vi "Client Tests.vi"() -> ()   [LabVIEW 2025]
uses:
  controls/Clint States Tests.ctl
  5TR Lab/5TR Lab/Global Variables/cRIO channels Input.vi
  5TR Lab/5TR Lab/Global Variables/General Glob.vi
panel:
  in  "Seek Forward Button":bool
  in  "Tab Control 3":T1(tab)
  in  "Cluster":T2
  in  "Cluster 2":T3
  in  "ID_HEATER_Stage_3 2":bool
  in  "ID_HEATER_Stage_2 2":bool
  in  "OD_HEATER_Stage_1":bool
  in  "ID_HEATER_Stage_3":bool
  in  "ID_HEATER_Stage_2":bool
  in  "Cluster 3":T4
  in  "AUX Chiller Pump_ 2":bool
  in  "AUX Chiller Pump_1":bool
  in  "Hc0 2":i32(listbox)
  out "Type Of Test":string
  in  "Add paramter":bool
  in  "Hc0":i32(listbox)
  out "Temp\n(C)":T5 {"UUT Discharge temp" format="%0.2f"; "UUT Suction temp" format="%0.2f"; "UUT Liquid temp" format="%0.2f"}
  out "Pressures\n(Mpa)":T6 {"UUT Discharge Pressure" format="%0.2f"; "UUT Suction Pressure" format="%0.2f"; "UUT Liquid Pressure" format="%0.2f"}
  in  "Tab Control":enum32{"Water Side capacity", "Page 2"}(tab)
  in  "Tab Control 2":T7(tab)
  out "WFR":dbl format="%0.2f"
  out "WPD":dbl format="%0.2f"
  out "T. Diff":dbl format="%0.2f"
  out "LWT":dbl format="%0.2f"
  out "EWT":dbl format="%0.2f"
  out "Running 3":bool
  out "Water Capacity":dbl format="%0.2f"
  out "Latent Capacity":dbl format="%0.2f"
  out "Sensible Capacity":dbl format="%0.2f"
  out "ID Entering WB":dbl format="%0.2f"
  out "ID Entering DB":dbl format="%0.2f"
  out "ID Leaving WB":dbl format="%0.2f"
  out "ID Leaving DB":dbl format="%0.2f"
  out "Air Capacity W":dbl format="%0.1f"
  out "Running 2":bool
  out "HB 2":dbl format="%0.2f"
  out "Running":bool
  out "Heat Balance %":dbl format="%0.1f"
  out "SC":dbl format="%0.2f"
  out "SH":dbl format="%0.2f"
  out "UUT Liquid Pressure 2":dbl format="%0.2f"
  out "Running":bool
  in  "Refrigerant":enum16{"R407c", "R410a", "R134a", "R22", ""}(ring)
  in  "Running Tests":string[](array[string])
  out "Total Capacity ID":dbl format="%0.2f"
  out "Total Capacity OD":dbl format="%0.2f"
  out "HB":dbl format="%0.2f"
  out "ID WFR":dbl format="%0.1f"
  out "result":dbl
  # "Sensor I/P Readings"
  # "Sensor O/P Values"
  # "W/W"
  # "Total Capacity\nWater-Side"
  # "C"
  # "C"
  # "C"
  # "gpm"
  # "Psi"
  # "Total Capacity\n Air-Side"
  # "DBT"
  # "WBT"
  # "Return"
  # "Supply"
  # "W"
  # "W"
  # "W"
  # "%"
  # "Thermal Transmittance"
  # "Thermal Bridging"
  # "Refrigerant"
  # "C"
  # "C"
  # "Ref Capacity"
  # "W"
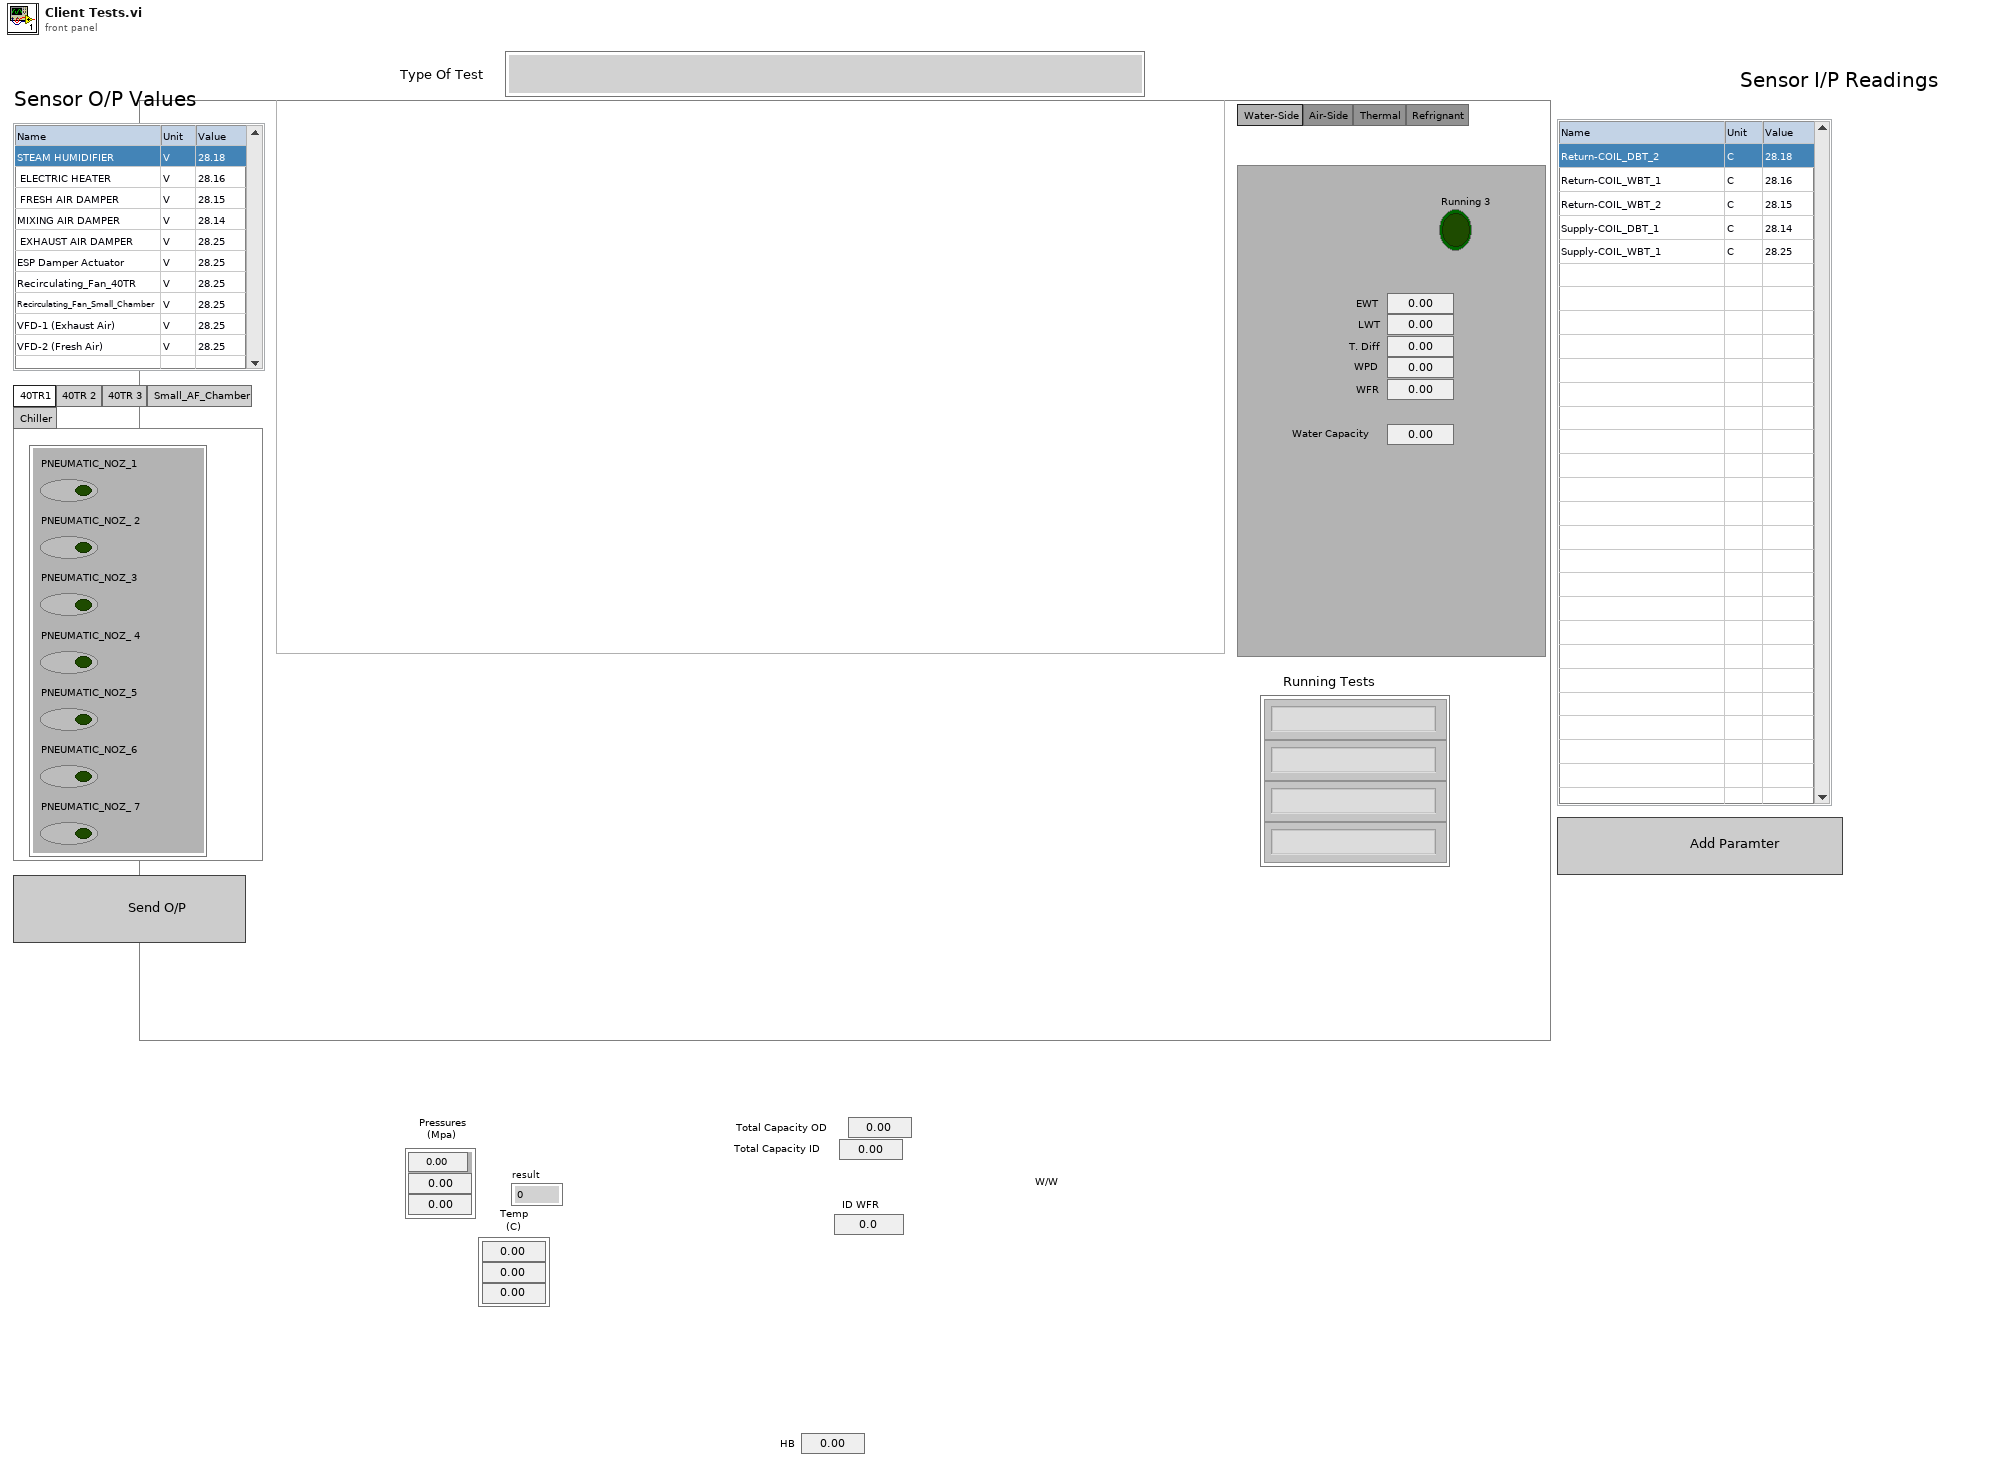
[diagram p1: front panel]
types:
  T1 = enum32{"40TR1", "40TR 2", "40TR 3", "Small_AF_Chamber", "Chiller"}
  T2 = cluster{"PNEUMATIC_NOZ_1":bool, "PNEUMATIC_NOZ_ 2":bool, "PNEUMATIC_NOZ_3":bool, "PNEUMATIC_NOZ_ 4":bool, "PNEUMATIC_NOZ_5":bool, "PNEUMATIC_NOZ_6":bool, "PNEUMATIC_NOZ_ 7":bool}
  T3 = cluster{"Recirculating_Fan_40TR":bool, "Recirculating_Fan_40TR 2":bool, "STEAM HUMIDIFIER":bool, "VFD-2 (Exahust Air)":bool, "VFD-2 (Fresh Air) ":bool, "VFD_Fan_Leak_setup":bool, "ID_HEATER_Stage_1":bool}
  T4 = cluster{"PNEUMATIC_NOZ_1":bool, "PNEUMATIC_NOZ_ 2":bool, "PNEUMATIC_NOZ_3":bool, "PNEUMATIC_NOZ_ 4":bool, "PNEUMATIC_NOZ_5":bool}
  T5 = cluster{"UUT Liquid temp":dbl, "UUT Suction temp":dbl, "UUT Discharge temp":dbl}
  T6 = cluster{"UUT Liquid Pressure":dbl, "UUT Suction Pressure":dbl, "UUT Discharge Pressure":dbl}
  T7 = enum32{"Water-Side", "Air-Side", "Thermal", "Refrignant"}
  T8 = typedef "Clint States Tests.ctl" = enum16{"Initialize", "Water Side", "Sensible capacity", "AIR SIDE Capacity", "Refrigrator Capacity"}
  T9 = cluster{"Room DP":dbl, "Barometric Pressure":dbl, "ID Nozzle DP":dbl, "OD Nozzle DP":dbl, "OD UUT Discharge Pressure":dbl, "OD UUT Suction Pressure":dbl, "OD UUT Liquid Pressure":dbl, "ID Humidifier Weight ":dbl, "ID UUT Condensate Weight":dbl, "ID Coil Condensate Weight":dbl, "OD Coil Water flow rate":dbl, "ID Flow Meter Channel":dbl}
  T10 = cluster{"ID UUT inlet DBT":dbl, "ID UUT inlet WBT":dbl, "ID UUT Outlet DBT":dbl, "OD UUT Outlet DBT":dbl, "ID UUT OUTLET WBT":dbl, "OD UUT INLET DBT":dbl, "OD UUT INLET WBT":dbl, "ID_EWT":dbl, "ID_LWT":dbl, "ID_Nozz_Temp":dbl}
  T11 = cluster{"ESP":dbl, "SP":dbl, "DP":dbl, "FCU WFR":dbl, "FCU Water PD":dbl, "RFM (lb/h)":dbl}
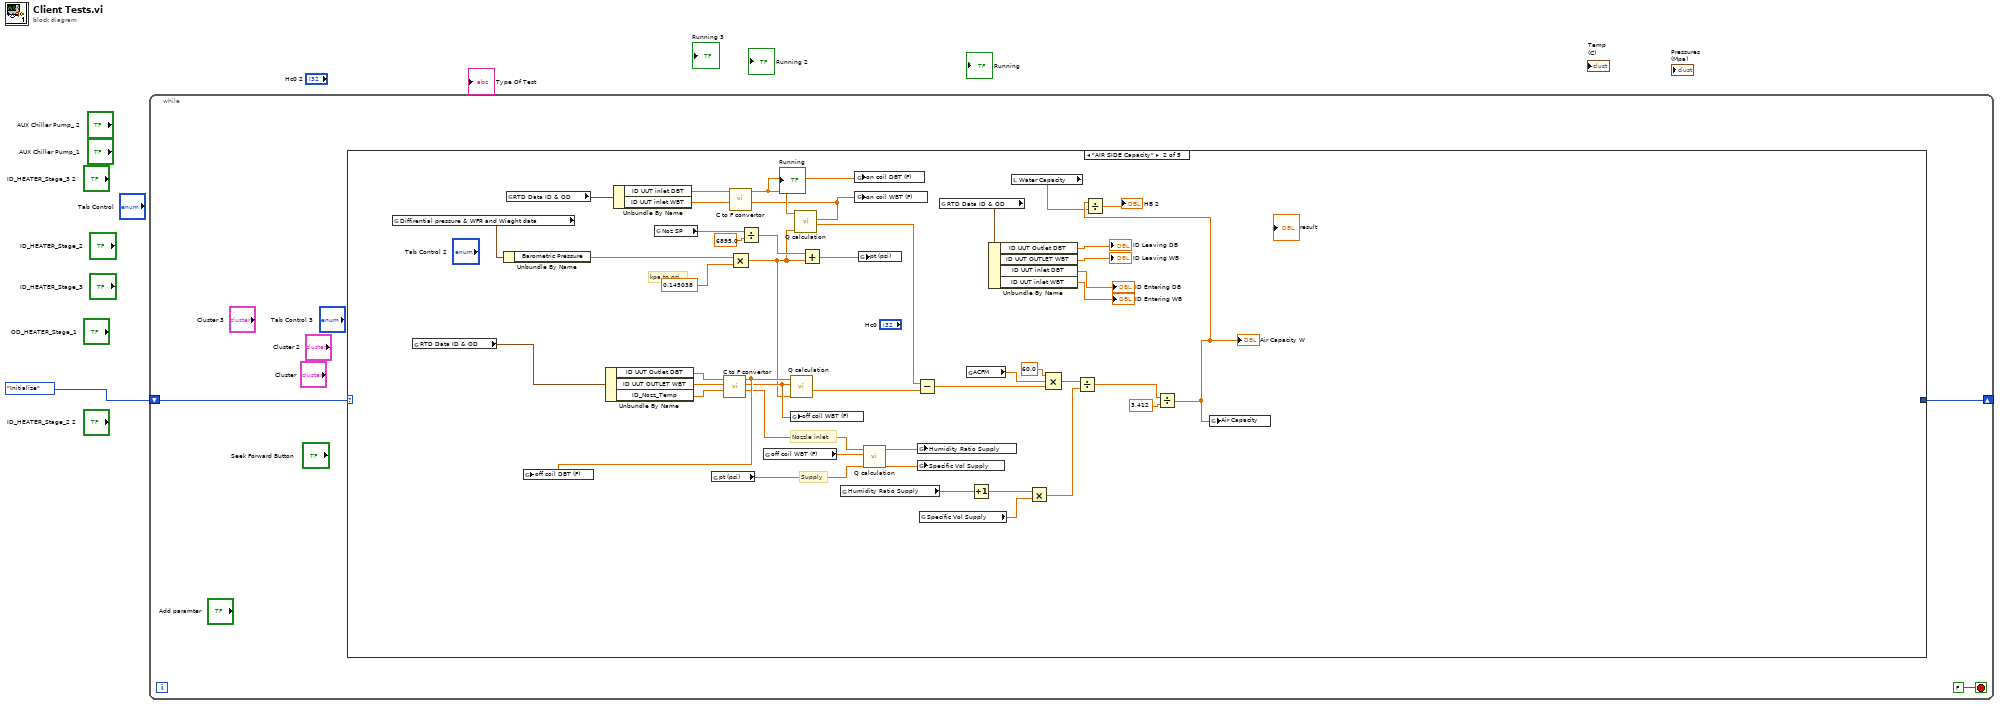
[diagram p0: block diagram]
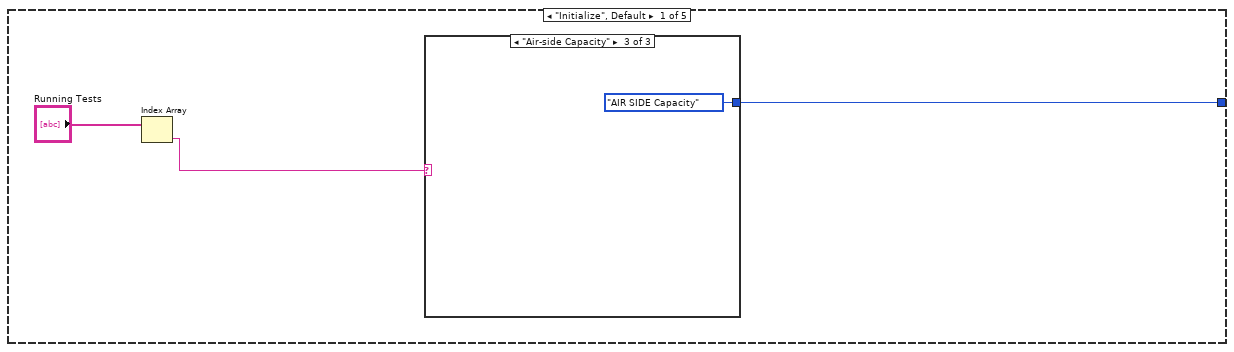
[diagram p2: hidden frame]
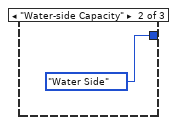
[diagram p4: hidden frame]
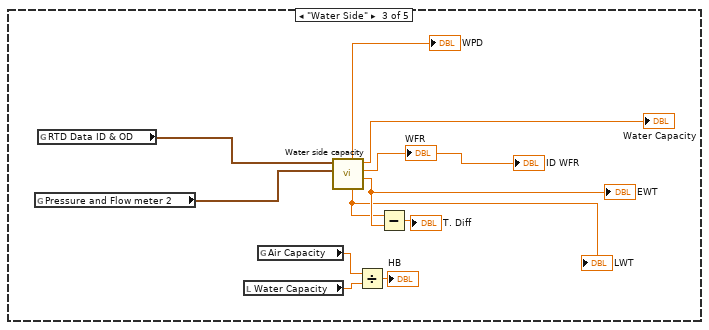
[diagram p5: hidden frame]
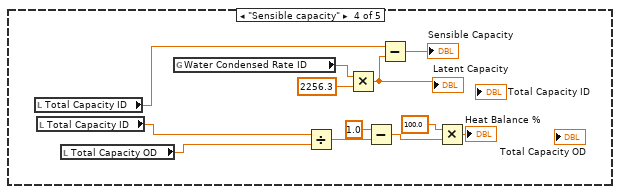
[diagram p6: hidden frame]
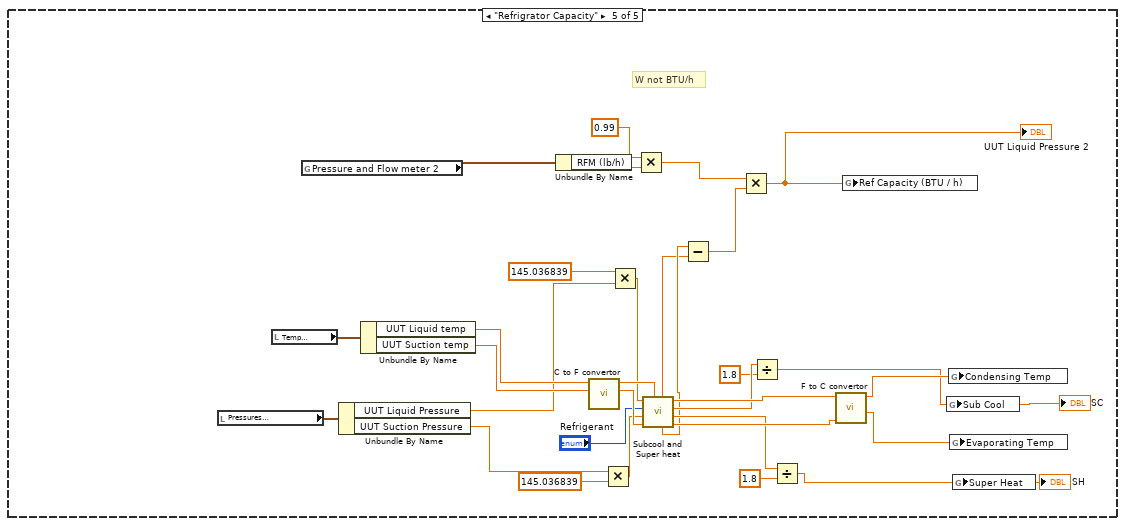
[diagram p7: hidden frame]
diagram:
  n1 = while {
    shift-right: [w2] -> _
    shift-left: Clint_States_Tests."Initialize" -> [w3]
    stop <- FALSE stop-if-true
    n2 = case shown="\"AIR SIDE Capacity\"" w3 {
      tunnel: [w7 _ _ _ _] -> w2
      frame "Initialize", Default {
        n3 = Index Array(array="Running Tests") -> (element=w5:string)  [unwired: 1 in]
        n4 = case shown="\"Air-side Capacity\"" w5 {
          tunnel: [_ Clint_States_Tests."Water Side" Clint_States_Tests."AIR SIDE Capacity"] -> w7
          frame "False", Default {
          }
          frame "Water-side Capacity" {
          }
          frame "Air-side Capacity" {
          }
        }
      }
      frame "AIR SIDE Capacity" {
        # "kpa to psi"
        # "Nozzle inlet"
        # "Supply"
        n5 = global read "cRIO channels Input.vi" "Diffirential pressure & WFR and Wieght data"() -> (w51:T9)
        n6 = global read "cRIO channels Input.vi" "RTD Data ID & OD"() -> (w53:T10)
        n7 = Unbundle By Name(w51) -> ("Barometric Pressure"=w50:dbl)
        n8 = global read "cRIO channels Input.vi" "RTD Data ID & OD"() -> (w52:T10)
        n9 = Unbundle By Name(w53) -> ("ID UUT Outlet DBT"=w38:dbl, "ID UUT OUTLET WBT"=w37:dbl, "ID_Nozz_Temp"=w36:dbl)
        n10 = Unbundle By Name(w52) -> ("ID UUT inlet DBT"=w40:dbl, "ID UUT inlet WBT"=w39:dbl)
        n11 = global read "General Glob.vi" "Noz SP"() -> (w33:dbl)
        n12 = global read "General Glob.vi" "pt (psi)"() -> (w23:dbl)
        n13 = call "C to F convertor.vi"("Temp(C) 3"=w36, "Temp(C) 2"=w37, "Temp(C)"=w38) -> ("Temp (F) 3"=w25:dbl, "Temp (F) 2"=w27:dbl, "Temp (F)"=w28:dbl)  [unwired: 5 in, 1 out]
        n14 = global write "General Glob.vi" "off coil DBT (F)"(w28) -> ()
        n15 = call "C to F convertor.vi"("Temp(C) 3"=w39, "Temp(C)"=w40) -> ("Temp (F) 3"=w29:dbl, "Temp (F)"=w30:dbl)  [unwired: 6 in, 2 out]
        n16 = Multiply(x=w50, y=0.145038) -> (x*y=w26:dbl)
        n17 = Divide(x=w33, y=6895.0) -> (x/y=w32:dbl)
        n18 = global read "General Glob.vi" "off coil WBT (F)"() -> (w24:dbl)
        n19 = call "Q calculation.vi"("Presure psi"=w26, "WB Temp"=w27, "DB Temp"=w28) -> ("Enthalpy"=w19:dbl)  [unwired: 5 in, 3 out]
        n20 = global write "General Glob.vi" "off coil WBT (F)"(w27) -> ()
        n21 = call "Q calculation.vi"("Presure psi"=w26, "WB Temp"=w29, "DB Temp"=w30) -> ("Enthalpy"=w20:dbl)  [unwired: 5 in, 3 out]
        n22 = Add(x=w32, y=w26) -> (x+y=w31:dbl)
        n23 = global read "General Glob.vi" "Humidity Ratio Supply"() -> (w44:dbl)
        n24 = global write "General Glob.vi" "on coil DBT (F)"(w30) -> ()
        n25 = global write "General Glob.vi" "on coil WBT (F)"(w29) -> ()
        n26 = global write "General Glob.vi" "pt (psi)"(w31) -> ()
        n27 = call "Q calculation.vi"("Presure psi"=w23, "WB Temp"=w24, "DB Temp"=w25) -> ("Specific Volume"=w21:dbl, "Humidty Ratio"=w22:dbl)  [unwired: 5 in, 2 out]
        n28 = Subtract(x=w20, y=w19) -> (x-y=w46:dbl)
        n29 = global write "General Glob.vi" "Humidity Ratio Supply"(w22) -> ()
        n30 = global write "General Glob.vi" "Specific Vol Supply"(w21) -> ()
        n31 = global read "General Glob.vi" "Specific Vol Supply"() -> (w42:dbl)
        n32 = global read "cRIO channels Input.vi" "RTD Data ID & OD"() -> (w17:T10)
        n33 = global read "General Glob.vi" "ACFM"() -> (w47:dbl)
        n34 = Increment(x=w44) -> (x+1=w43:dbl)
        n35 = Unbundle By Name(w17) -> ("ID UUT Outlet DBT"=→"ID Leaving DB":dbl, "ID UUT OUTLET WBT"=→"ID Leaving WB":dbl, "ID UUT inlet DBT"=→"ID Entering DB":dbl, "ID UUT inlet WBT"=→"ID Entering WB":dbl)
        n36 = local read "Water Capacity"() -> (w11:dbl)
        n37 = Multiply(x=w43, y=w42) -> (x*y=w41:dbl)
        n38 = Compound Arithmetic op=MULTIPLY(60.0 ("value"), w47, w46) -> (w45:dbl)
        n39 = Divide(x=w45, y=w41) -> (x/y=w18:dbl)
        n40 = Divide(x=w18, y=3.412) -> (x/y=w12:dbl)
        "Air Capacity W" <- w12
        n41 = Divide(x=w12, y=w11) -> (x/y=→"HB 2":dbl)
        n42 = global write "General Glob.vi" "Air Capacity"(w12) -> ()
      }
      frame "Water Side" {
        n43 = global read "cRIO channels Input.vi" "Pressure and Flow meter 2"() -> (w63:T11)
        n44 = global read "cRIO channels Input.vi" "RTD Data ID & OD"() -> (w64:T10)
        n45 = local read "Water Capacity"() -> (w59:dbl)
        n46 = global read "General Glob.vi" "Air Capacity"() -> (w54:dbl)
        n47 = call "Water side capacity.vi"("Pressure and Flow meter in"=w63, "RTD Data ID & OD"=w64) -> ("FCU EWT"=w56:dbl, "FCU WFR 2"=→"ID WFR" →"WFR":dbl, "WCC"=→"Water Capacity":dbl, "FCU LWT"=w55:dbl, "FCU Water PD 2"=→"WPD":dbl)  [unwired: 5 in]
        "EWT" <- w56
        "LWT" <- w55
        n48 = Divide(x=w54, y=w59) -> (x/y=→"HB":dbl)
        n49 = Subtract(x=w55, y=w56) -> (x-y=→"T. Diff":dbl)
      }
      frame "Sensible capacity" {
        n50 = local read "Total Capacity ID"() -> (w65:dbl)
        n51 = local read "Total Capacity ID"() -> (w67:dbl)
        n52 = local read "Total Capacity OD"() -> (w66:dbl)
        n53 = global read "cRIO channels Input.vi" "Water Condensed Rate ID"() -> (w75:dbl)
        n54 = Divide(x=w67, y=w66) -> (x/y=w71:dbl)
        n55 = Multiply(x=w75, y=2256.3) -> (x*y=w68:dbl)
        "Latent Capacity" <- w68
        n56 = Subtract(x=1.0, y=w71) -> (x-y=w70:dbl)
        n57 = Subtract(x=w65, y=w68) -> (x-y=→"Sensible Capacity":dbl)
        n58 = Multiply(x=100.0, y=w70) -> (x*y=→"Heat Balance %":dbl)
      }
      frame "Refrigrator Capacity" {
        # "W not BTU/h"
        n59 = local read "Pressures\n(Mpa)"() -> (w106:T6)
        n60 = local read "Temp\n(C)"() -> (w107:T5)
        n61 = global read "cRIO channels Input.vi" "Pressure and Flow meter 2"() -> (w87:T11)
        n62 = Unbundle By Name(w106) -> ("UUT Liquid Pressure"=w77:dbl, "UUT Suction Pressure"=w100:dbl)
        n63 = Unbundle By Name(w107) -> ("UUT Liquid temp"=w105:dbl, "UUT Suction temp"=w103:dbl)
        n64 = Unbundle By Name(w87) -> ("RFM (lb/h)"=w85:dbl)
        n65 = call "C to F convertor.vi"("Temp(C) 2"=w103, "Temp(C)"=w105) -> ("Temp (F) 2"=w102:dbl, "Temp (F)"=w104:dbl)  [unwired: 6 in, 2 out]
        n66 = Multiply(x=w100, y=145.036839) -> (x*y=w98:dbl)
        n67 = Multiply(x=145.036839 ("y"), y=w77) -> (x*y=w99:dbl)
        n68 = Multiply(x=0.99 ("y"), y=w85) -> (x*y=w84:dbl)
        n69 = call "Subcool and Super heat.vi"("LLT"=w104, "SLT"=w102, "SLP"=w98, "Refrigerant"="Refrigerant", "LLP"=w99) -> ("SupperHeat 2"=w94:dbl, "Evaporating Temp"=w89:dbl, "Sub-Cooling"=w92:dbl, "Condensing Temp"=w96:dbl, "Enth_Vap"=w83:dbl, "Enth_Liq"=w82:dbl)  [unwired: 1 in]
        n70 = Subtract(x=w83, y=w82) -> (x-y=w81:dbl)
        n71 = Multiply(x=w84, y=w81) -> (x*y=w80:dbl)
        "UUT Liquid Pressure 2" <- w80
        n72 = Divide(x=w92, y=1.8) -> (x/y=w79:dbl)
        "SC" <- w79
        n73 = Divide(x=w89, y=1.8) -> (x/y=w88:dbl)
        "SH" <- w88
        n74 = call "F to C convertor.vi"("Temp(F) 4"=w94, "Temp(F)"=w96) -> ("Temp (C) 3"=w93:dbl, "Temp (C)"=w95:dbl)  [unwired: 6 in, 2 out]
        n75 = global write "General Glob.vi" "Ref Capacity (BTU / h)"(w80) -> ()
        n76 = global write "General Glob.vi" "Sub Cool"(w79) -> ()
        n77 = global write "General Glob.vi" "Condensing Temp"(w95) -> ()
        n78 = global write "General Glob.vi" "Evaporating Temp"(w93) -> ()
        n79 = global write "General Glob.vi" "Super Heat"(w88) -> ()
      }
    }
  }
